vi "Main Page.vi"(8 "error in (no error)":errorcluster, 11 "Node Ptr":T1 format="%.0x") -> (0 "error out":errorcluster)   [LabVIEW 2020, in "SLSC Switch System Explorer.lvlib"]
uses:
  SLSC Switch System Explorer.lvlib
  <vilib>/NI VeriStand/Custom Device API/Custom Device Item Ref.ctl
  Main Page Controls.ctl
  <vilib>/NI VeriStand/Custom Device API/Custom Device API.lvlib
  Scripting/SLSC Switch Scripting.lvlib
panel:
  out "Reservation Group":string
  in  "Topology":string(combo)
  out "Model Number":string
  in  "SHDocVw.IWebBrowser":refnum<k7>(container)
  in  "Description":string
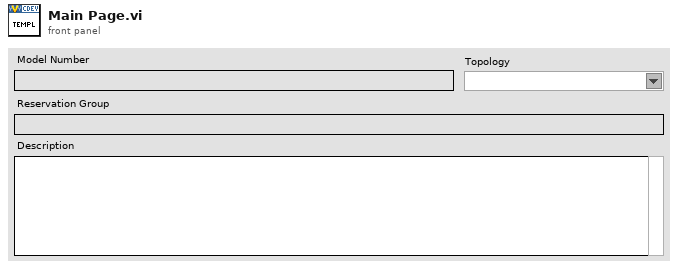
[diagram p1: front panel]
types:
  T1 = typedef "Custom Device API.lvlib/Custom Device Item Ref.ctl" = u64
  T2 = typedef "SLSC Switch System Explorer.lvlib/Main Page Controls.ctl" = cluster{"Description":refnum<vi>, "Model Number":refnum<vi>, "Topology":refnum<vi>, "Reservation Group":refnum<vi>}
  T3 = typedef "Custom Device API.lvlib/Custom Device Commands.ctl" = enum16{"Default", "Item renamed", "Shutdown", "Dynamic button pressed"}
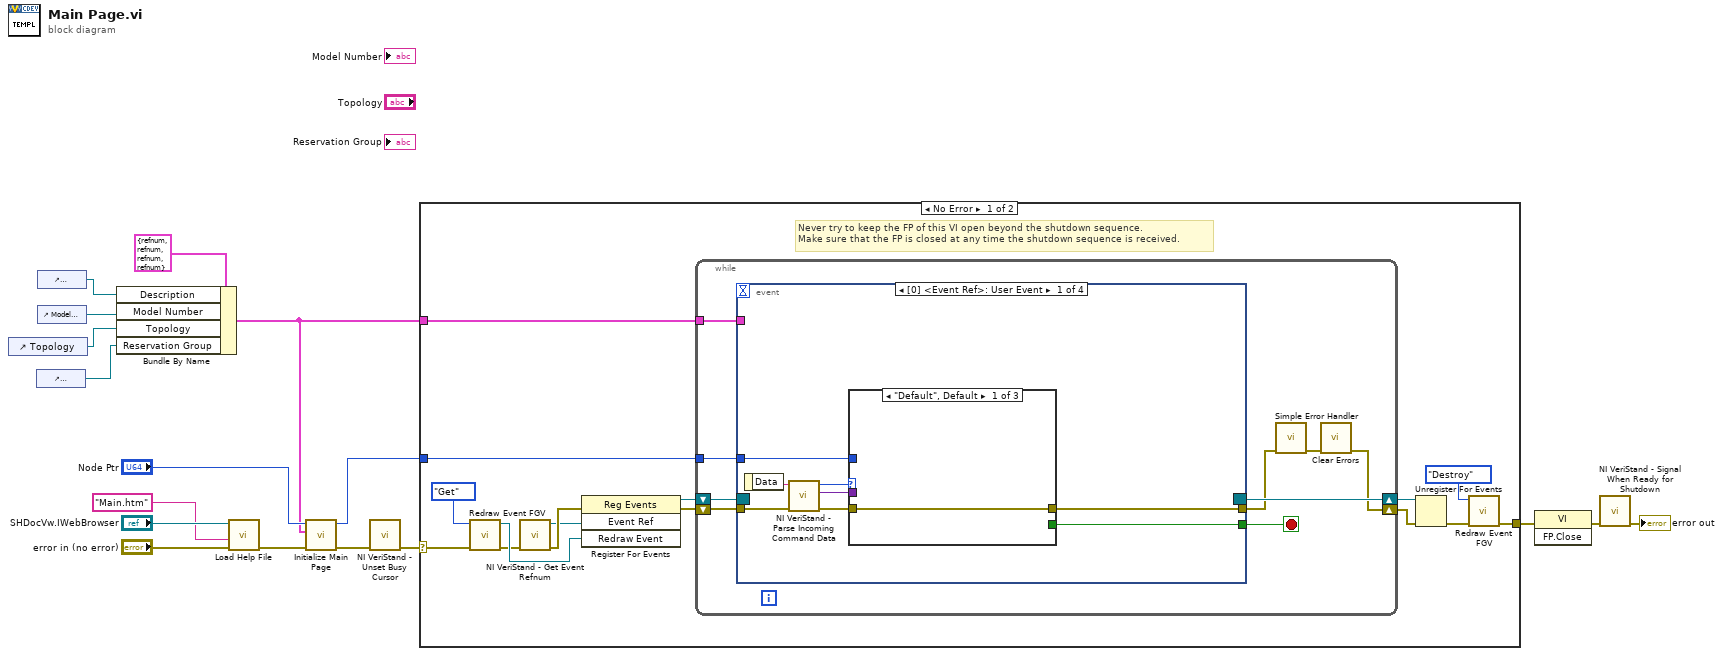
[diagram p0: block diagram]
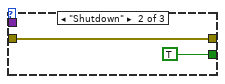
[diagram p2: hidden frame]
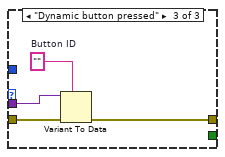
[diagram p3: hidden frame]
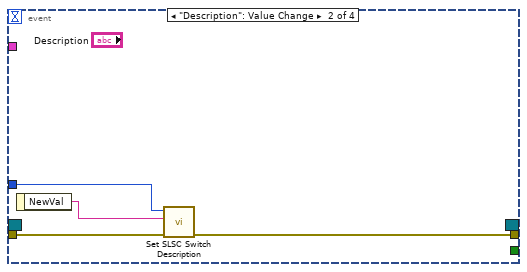
[diagram p4: hidden frame]
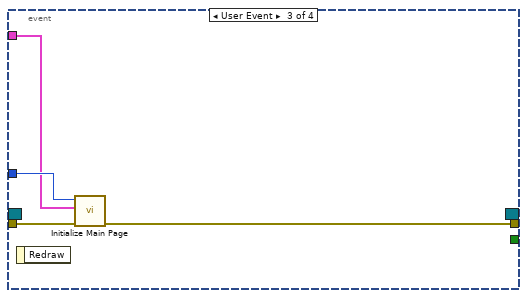
[diagram p5: hidden frame]
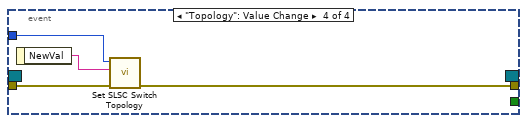
[diagram p6: hidden frame]
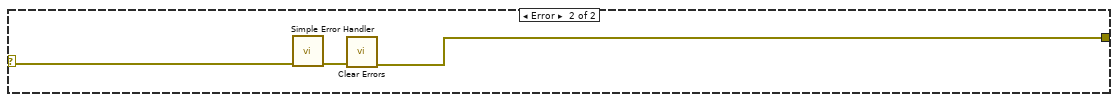
[diagram p7: hidden frame]
diagram:
  n1 = control-ref of="Topology"() -> (w4:refnum<vi>)
  n2 = control-ref of="Reservation Group"() -> (w1:refnum<vi>)
  n3 = control-ref of="Description"() -> (w7:refnum<vi>)
  n4 = control-ref of="Model Number"() -> (w3:refnum<vi>)
  n5 = Bundle By Name(cluster=T2 {"Description"=refnum, "Model Number"=refnum, "Topology"=refnum, "Reservation Group"=refnum} ("Main Page Controls"), "Description"=w7, "Model Number"=w3, "Topology"=w4, "Reservation Group"=w1) -> (w2:T2)
  n6 = call "Load Help File.vi"("error in (no error)"="error in (no error)", "HTML File to Load"="Main.htm" ("HTML File"), "Browser"="SHDocVw.IWebBrowser") -> ("error out"=w5:errorcluster)  [unwired: 8 in]
  n7 = call "Initialize Main Page.vi"("error in (no error)"=w5, "Main Page Controls"=w2, "Item Ref in"="Node Ptr") -> ("error out"=w13:errorcluster, "Item Ref out"=w10:T1)  [unwired: 7 in]
  n8 = call <vilib>:"NI VeriStand - Unset Busy Cursor.vi"("error in (no error)"=w13) -> ("error out"=w12:errorcluster)  [unwired: 10 out]
  n9 = case shown="No Error" w12 {
    selector: w12 -> [w20 w71]
    tunnel: [w22 w69] -> w17
    tunnel: w10 -> [w26 _]
    tunnel: w2 -> [w24 _]
    frame No Error {
      # "Never try to keep the FP of this VI open beyond the shutdown sequence.\nMake sure that the FP is closed at any time the shutdown sequence is received."
      n10 = call "Redraw Event FGV.vi"("error in (no error)"=w20, "Action (Get)"=enum16{"Get", "Destroy"}."Get") -> ("error out"=w19:errorcluster, "Redraw Event"=w25:refnum<user-event>)  [unwired: 8 in]
      n11 = call <vilib>:"NI VeriStand - Get Event Refnum.vi"("error in (no error)"=w19) -> ("error out"=w32:errorcluster, "Event Ref"=w29:refnum<user-event>)  [unwired: 9 out]
      n12 = register-events(error in=w32, w29, w25) -> (reference out=w27:refnum<event-registration>, error out=w28:errorcluster)  [unwired: 1 in]
      n13 = while {
        tunnel: w26 -> [w37]
        shift-right: [w34] -> w30
        shift-left: w28 -> [w40]
        shift-right: [w41] -> w31
        shift-left: w27 -> [w39]
        tunnel: w24 -> [w33]
        stop <- w38 stop-if-true
        n14 = event shown="[0] <Event Ref>: User Event" {
          selector: w39 -> [_ _ _ _]
          dyn-events: [_ _ _ _] -> w41
          timeout: _ -> [_ _ _ _]
          tunnel: w40 -> [w49 w59 w62 w68]
          tunnel: [w45 _ _ _] -> w38
          tunnel: [w44 w58 w61 w67] -> w36
          tunnel: w37 -> [w43 w60 w64 w66]
          tunnel: w33 -> [_ _ w63 _]
          event User Event {
            n15 = event-data() -> ("Data"=w48:string)  [unwired: 1 out]
            n16 = call <vilib>:"NI VeriStand - Parse Incoming Command Data.vi"("error in (no error)"=w49, "Incoming data"=w48) -> ("error out"=w47:errorcluster, "Outgoing data"=w42:variant, "Action"=w46:T3)  [unwired: 7 out]
            n17 = case shown="\"Default\", Default" w46 {
              tunnel: w47 -> [w50 w51 w56]
              tunnel: [_ TRUE _] -> w45
              tunnel: [w50 w51 w53] -> w44
              tunnel: w43 -> [_ _ _]
              tunnel: w42 -> [_ _ w55]
              frame "Default", Default {
              }
              frame "Shutdown" {
              }
              frame "Dynamic button pressed" {
                w54 = ""  # Button ID
                n18 = Variant To Data(error in=w56, type=w54, Variant=w55) -> (error out=w53:errorcluster)  [unwired: 1 out]
              }
            }
          }
          event "Description": Value Change {
            n19 = event-data() -> ("NewVal"=w57:string)  [unwired: 1 out]
            n20 = call "Set SLSC Switch Description.vi"("error in"=w59, "description"=w57, "slsc switch custom device in"=w60) -> ("error out"=w58:errorcluster)  [unwired: 7 in, 1 out]
          }
          event User Event {
            n21 = event-data() -> ()  [unwired: 2 out]
            n22 = call "Initialize Main Page.vi"("error in (no error)"=w62, "Main Page Controls"=w63, "Item Ref in"=w64) -> ("error out"=w61:errorcluster)  [unwired: 7 in, 1 out]
          }
          event "Topology": Value Change {
            n23 = event-data() -> ("NewVal"=w65:string)  [unwired: 1 out]
            n24 = call "Set SLSC Switch Topology.vi"("error in"=w68, "topology"=w65, "slsc switch custom device in"=w66) -> ("error out"=w67:errorcluster)  [unwired: 7 in, 1 out]
          }
        }
        n25 = call <vilib>:"Simple Error Handler.vi"("error in (no error)"=w36) -> ("error out"=w35:errorcluster)  [unwired: 1 in, 7 out]
        n26 = call <vilib>:"Clear Errors.vi"("error in (no error)"=w35) -> ("error out"=w34:errorcluster)  [unwired: 1 in, 5 out]
      }
      n27 = Unregister For Events(event registration refnum=w31, error in=w30) -> (error out=w23:errorcluster)
      n28 = call "Redraw Event FGV.vi"("error in (no error)"=w23, "Action (Get)"=enum16{"Get", "Destroy"}."Destroy") -> ("error out"=w22:errorcluster)  [unwired: 8 in, 1 out]
    }
    frame Error {
      n29 = call <vilib>:"Simple Error Handler.vi"("error in (no error)"=w71) -> ("error out"=w70:errorcluster)  [unwired: 1 in, 7 out]
      n30 = call <vilib>:"Clear Errors.vi"("error in (no error)"=w70) -> ("error out"=w69:errorcluster)  [unwired: 1 in, 5 out]
    }
  }
  n31 = invoke class="VI" method="FP.Close"(error in=w17) -> (error out=w16:errorcluster)  [unwired: 2 in, 2 out]
  n32 = call <vilib>:"NI VeriStand - Signal When Ready for Shutdown.vi"("error in (no error)"=w16) -> ("error out"=→"error out":errorcluster)  [unwired: 10 out]
